vi "GDSAPI_CreateClass.vi"(7 "KeepLvClassRefOpen(False)":bool, 8 "error in (no error)":errorcluster, 9 "ClassIcon(Random colors are used if not wired)":T1, 10 "CreateClassType":T3={"ClassProvider"=enum."GOOP-3(By reference)", "NewClassFolder"=path "", "ParentLvClassFilePath"=path "", "ClassName"="", "ClassDescription"="", "ClassTemplate"=enum."Standard", "ParentInterfacesFilePath"=[]}, 11 "ProjectItemToCreateClassUnder":refnum<vi>) -> (0 "error out":errorcluster, 2 "LVClassLibraryRefnum":refnum<vi>, 3 "LvClassFileOut":path)   [LabVIEW 2020]
doc: "NOT Yet implemented"
uses:
  ClassProviders/Provider_LvNativeClass/ClassWriterNative_class/ClassWriterNative.lvclass
  ClassProviders/Provider_EndevoGOOP300/ClassWriterGOOP300_class/ClassWriterGOOP300.lvclass
  ClassProviders/Provider_EndevoGOOP400/ClassWriterGOOP400_class/ClassWriterGOOP400.lvclass
  ClassProviders/Provider_BaseClassInterface/CreateClassData.ctl
  ClassProviders/Provider_BaseClassInterface/ClassWriter_class/ClassWriter.lvclass
  ClassProviders/Common/ScriptingFunctions/Scripting_ConnectorPanePatternType.ctl
  ClassProviders/Common/LvIcon_class/GDSLvIcon_ClassColorTypes.ctl
  C:/VIT/GitHub/OpenGDS/resource/Framework/Providers/Open_GDS/ClassProviders/Provider_BaseClassInterface/ClassWriter_class/ClassWriter.lvclass
  C:/VIT/GitHub/OpenGDS/resource/Framework/Providers/Open_GDS/ClassProviders/Provider_LvNativeClass/ClassWriterNative_class/ClassWriterNative.lvclass
  C:/VIT/GitHub/OpenGDS/resource/Framework/Providers/Open_GDS/ClassProviders/Provider_EndevoGOOP300/ClassWriterGOOP300_class/ClassWriterGOOP300.lvclass
  C:/VIT/GitHub/OpenGDS/resource/Framework/Providers/Open_GDS/ClassProviders/Provider_EndevoGOOP400/ClassWriterGOOP400_class/ClassWriterGOOP400.lvclass
  GDSAPI_SubVIs/GDSAPI_ClassProviderType.ctl
  GDSAPI_CreateClassType.ctl
  GDSAPI_SubVIs/GDSAPI_ClassTemplateType.ctl
  GDSAPI_SubVIs/GDSAPI_ClassIcon.ctl
  GDSAPI_SubVIs/GDSAPI_ClassIconType.ctl
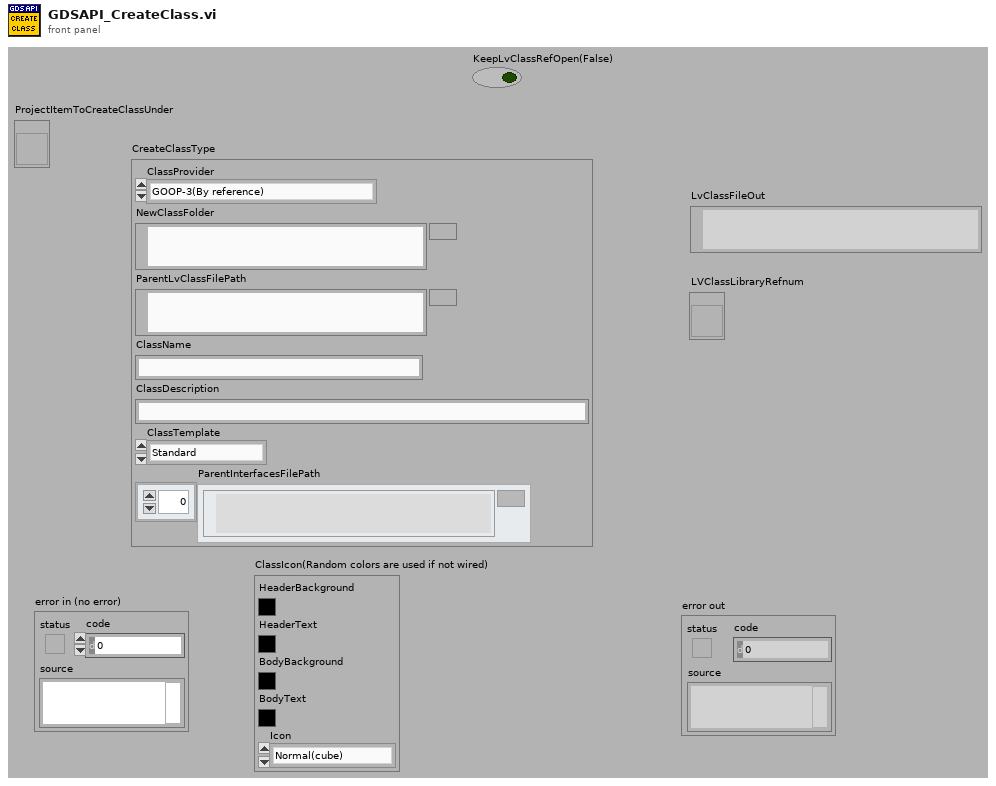
[diagram p1: front panel]
types:
  T1 = typedef "GDSAPI_ClassIcon.ctl" = cluster{"HeaderBackground":u32, "HeaderText":u32, "BodyBackground":u32, "BodyText":u32, "Icon":T2}
  T2 = typedef "GDSAPI_ClassIconType.ctl" = enum16{"Normal(cube)", "Actor", "Message", "Interface"}
  T3 = typedef "GDSAPI_CreateClassType.ctl" = cluster{"ClassProvider":T4, "NewClassFolder":path, "ParentLvClassFilePath":path, "ClassName":string, "ClassDescription":string, "ClassTemplate":T5, "ParentInterfacesFilePath":path[]}
  T4 = typedef "GDSAPI_ClassProviderType.ctl" = enum16{"LabVIEW Native(By value)", "GOOP-3(By reference)", "GOOP-4(By reference)"}
  T5 = typedef "GDSAPI_ClassTemplateType.ctl" = enum16{"Standard", "Singleton"}
  T6 = typedef "GDSLvIcon_ClassColorTypes.ctl" = cluster{"Frame":u32, "Header Text Color":u32, "Header Background":u32, "BodyBackgroundPublic":u32, "BodyBackgroundProtected":u32, "BodyBackgroundPrivate":u32, "Body Text Color":u32, "Frame thickness":u8, "ProtectedPrivateSame":bool, "Icon Header Size":u8, "Font Compression":enum16{"Auto", "On", "Off"}, "CapitalOnly":bool}
  T7 = cluster{"Colors":T6, "LibraryIcon":cluster{"LibraryIcon":string, "HeaderRows(1)":u8}}
  T8 = typedef "ClassWriter.lvclass/CreateClassData.ctl" = cluster{"ClassName":string, "ClassFolder":path, "ClassDescription":string, "ClassTemplateOptions":string, "BaseClass(ProjectStringPath or LvClassFilePath)":variant, "ExtraCreateParameters":variant, "FolderSuffix":string, "ParentInterfaces":path[]}
  T9 = typedef "Scripting_ConnectorPanePatternType.ctl" = u16
  T10 = typedef "GDSLvCLass_ClassSettingsType.ctl" = cluster{"ClassProviderName":string, "ClassTemplateUsed":string, "ClassTemplateVersion":string, "ClassDescription":string, "PlugIns":T11[], "ConnectorPanePattern":string}
  T11 = typedef "GDSLvClass_PlugIn.ctl" = cluster{"Type":T12, "ID":string, "Version":string, "Path":path, "Name":string, "Data":variant}
  T12 = typedef "GDSLvClass_PlugInTypes.ctl" = enum16{"DesignPattern", "MethodTypes"}
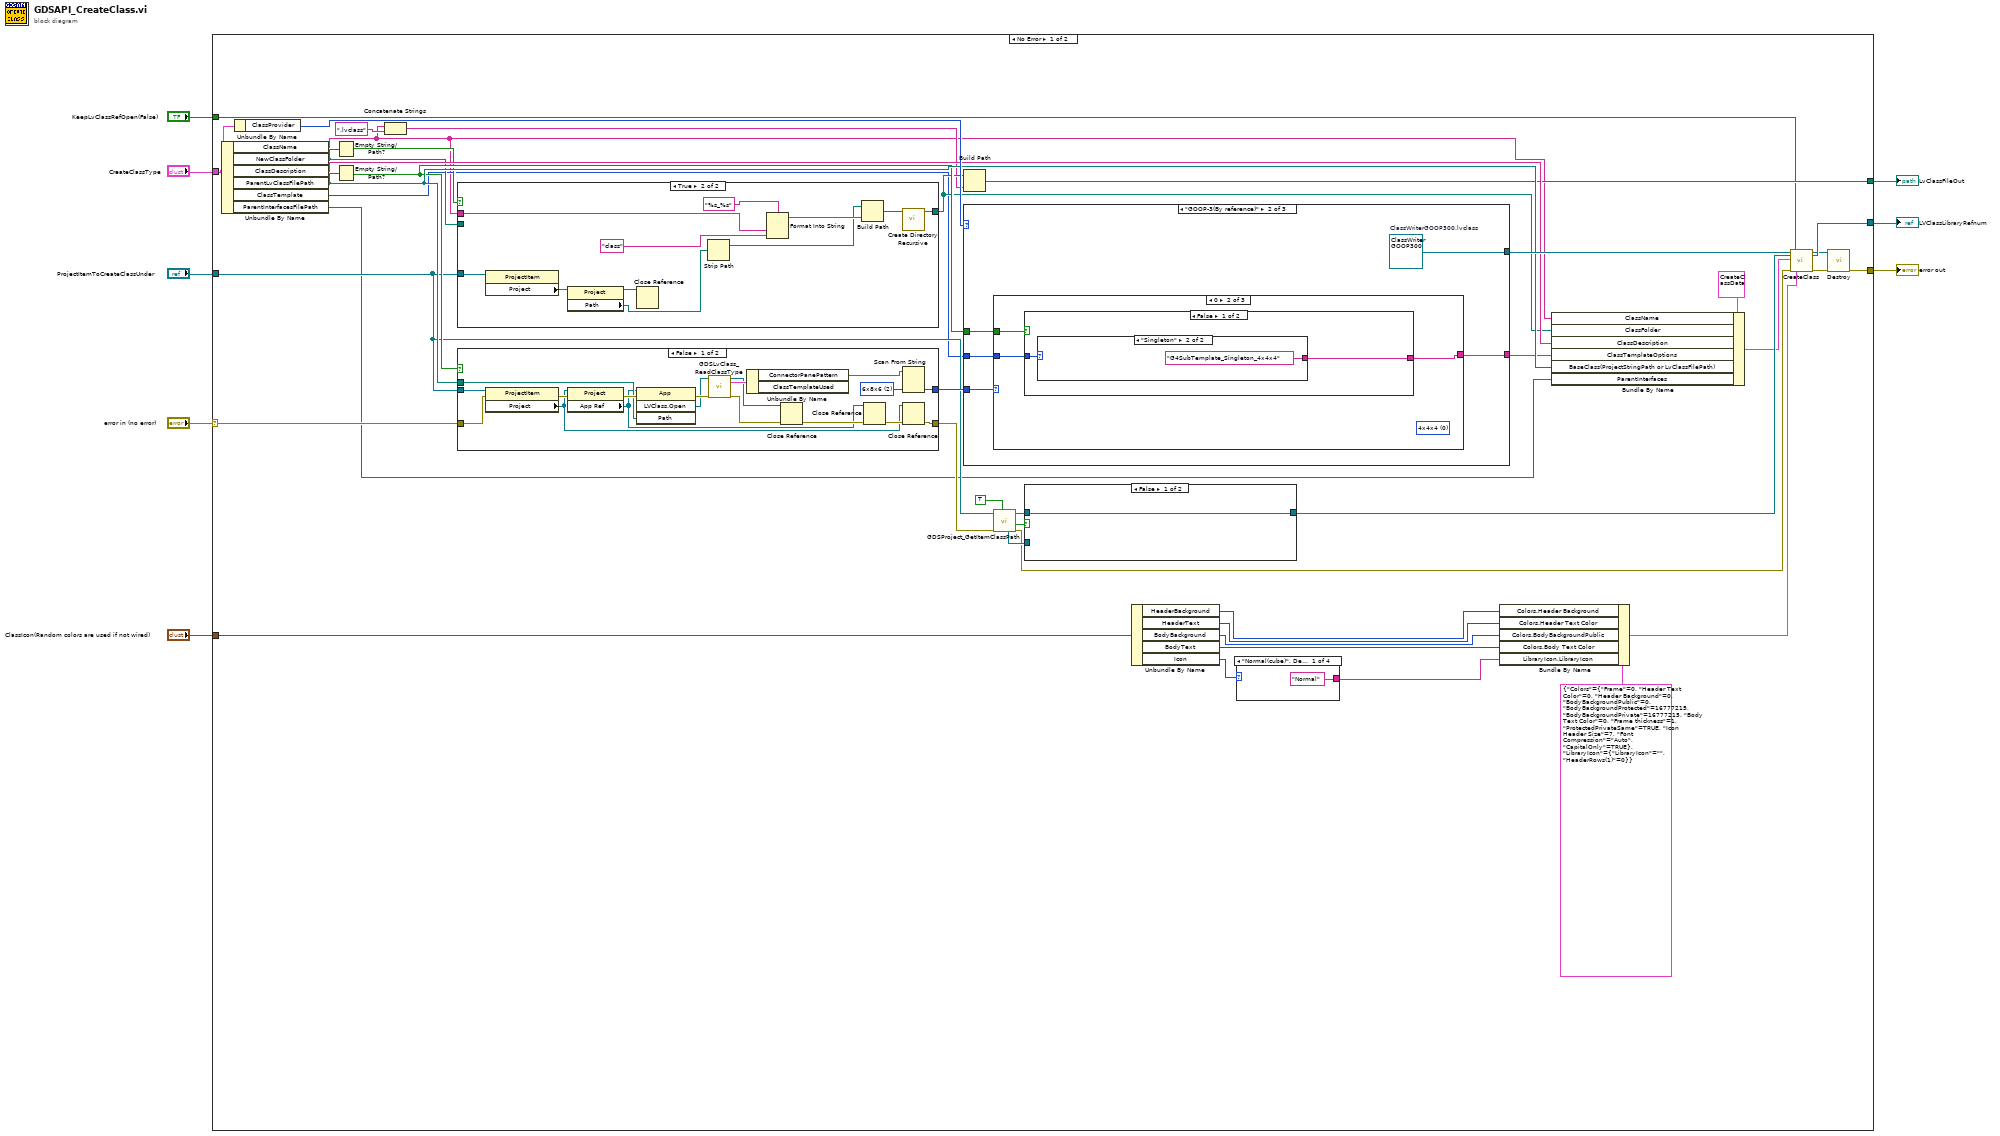
[diagram p0: block diagram]
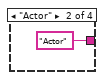
[diagram p2: hidden frame]
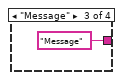
[diagram p3: hidden frame]
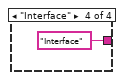
[diagram p4: hidden frame]
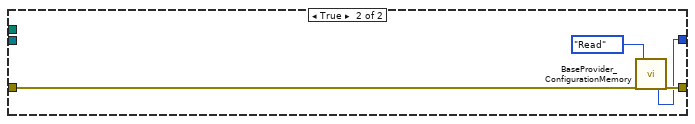
[diagram p6: hidden frame]
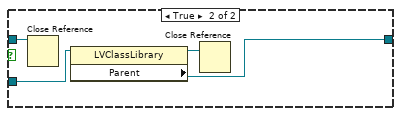
[diagram p7: hidden frame]
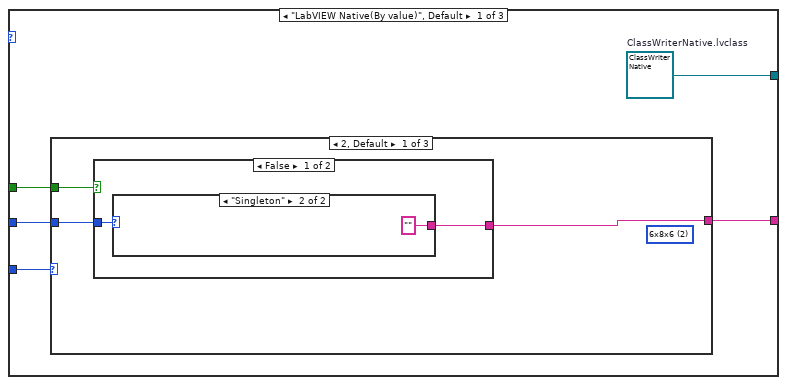
[diagram p8: hidden frame]
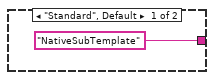
[diagram p9: hidden frame]
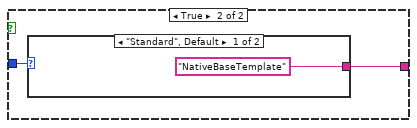
[diagram p10: hidden frame]
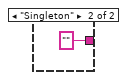
[diagram p11: hidden frame]
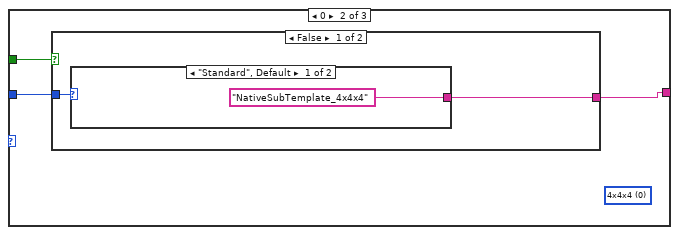
[diagram p12: hidden frame]
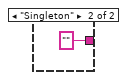
[diagram p13: hidden frame]
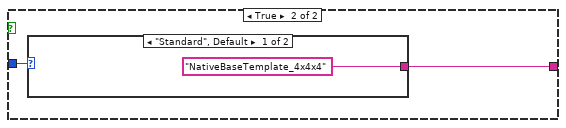
[diagram p14: hidden frame]
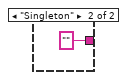
[diagram p15: hidden frame]
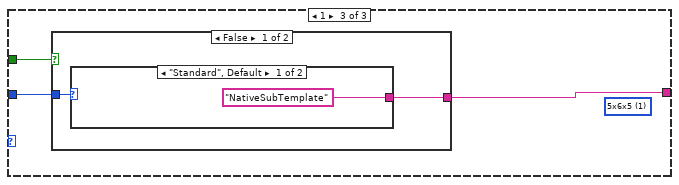
[diagram p16: hidden frame]
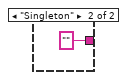
[diagram p17: hidden frame]
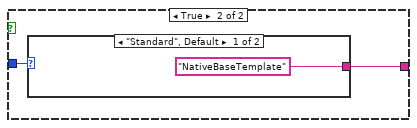
[diagram p18: hidden frame]
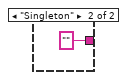
[diagram p19: hidden frame]
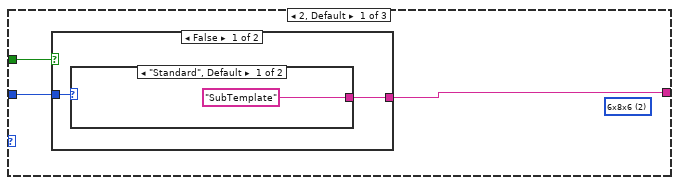
[diagram p20: hidden frame]
diagram:
  n1 = case shown="No Error" "error in (no error)" {
    selector: "error in (no error)" -> [w10 w208]
    tunnel: [w44 _] -> w8
    tunnel: [w40 w208] -> w7
    tunnel: "CreateClassType" -> [w38 _]
    tunnel: "ProjectItemToCreateClassUnder" -> [w29 _]
    tunnel: "ClassIcon(Random colors are used if not wired)" -> [w26 _]
    tunnel: [w16 _] -> w3
    tunnel: "KeepLvClassRefOpen(False)" -> [w11 _]
    frame No Error {
      n2 = Unbundle By Name(w38) -> ("ClassName"=w14:string, "NewClassFolder"=w30:path, "ClassDescription"=w37:string, "ParentLvClassFilePath"=w35:path, "ClassTemplate"=w15:T5, "ParentInterfacesFilePath"=w9:path[])
      n3 = Unbundle By Name(w38) -> ("ClassProvider"=w42:T4)
      n4 = Empty String/Path?(string/path=w30) -> (empty?=w31:bool)
      n5 = Empty String/Path?(string/path=w35) -> (empty?=w33:bool)
      n6 = Concatenate Strings(w14, ".lvclass" ("string")) -> (w17:string)
      n7 = case shown="True" w31 {
        tunnel: w30 -> [w55 _]
        tunnel: [w55 w58] -> w19
        tunnel: w29 -> [_ w66]
        tunnel: w14 -> [_ w56]
        frame False {
        }
        frame True {
          n8 = property class="ProjectItem"(reference=w66) -> ("Project"=w65:refnum<vi>)  [unwired: 1 in, 2 out]
          n9 = property class="Project"(reference=w65) -> (reference out=w63:refnum<vi>, "Path"=w64:path)  [unwired: 1 in, 1 out]
          n10 = Close Reference(reference=w63) -> ()  [unwired: 1 in, 1 out]
          n11 = Strip Path(path=w64) -> (stripped path=w59:path)  [unwired: 1 out]
          n12 = Format Into String(format string="%s_%s", w56, "class" ("format string")) -> (resulting string=w61:string)  [unwired: 2 in, 1 out]
          n13 = Build Path(base path=w59, name or relative path=w61) -> (appended path=w60:path)
          n14 = call <vilib>:"Create Directory Recursive.vi"("directory"=w60) -> ("directory copy"=w58:path)  [unwired: 4 in, 2 out]
        }
      }
      n15 = case shown="False" w33 {
        tunnel: [w67 w87] -> w36
        tunnel: [w81 w86] -> w34
        tunnel: w29 -> [w80 _]
        tunnel: w10 -> [w79 w85]
        tunnel: w35 -> [w74 _]
        frame False {
          w82 = T9 2 items=["4x4x4", "5x6x5", "6x8x6"] ("Pattern")
          n16 = property class="ProjectItem"(reference=w80, error in=w79) -> (error out=w78:errorcluster, "Project"=w69:refnum<vi>)  [unwired: 1 out]
          n17 = property class="Project"(reference=w69, error in=w78) -> (error out=w77:errorcluster, "App Ref"=w71:refnum<vi>)  [unwired: 1 out]
          n18 = invoke class="App" method="LVClass.Open"(reference=w71, error in=w77, "Path"=w74) -> (error out=w76:errorcluster, "LVClass.Open"=w75:refnum<vi>)  [unwired: 1 in, 2 out]
          n19 = call "GDSLvClass_ReadClassType.vi"("Class Refnum In"=w75, "error in (no error)"=w76) -> ("Class Refnum Out"=w73:refnum<vi>, "ClassSettings"=w84:T10, "error out"=w68:errorcluster)  [unwired: 15 in]
          n20 = Unbundle By Name(w84) -> ("ConnectorPanePattern"=w83:string)  [unwired: 1 out]
          n21 = Close Reference(reference=w73, error in (no error)=w68) -> (error out=w72:errorcluster)
          n22 = Close Reference(reference=w71, error in (no error)=w72) -> (error out=w70:errorcluster)
          n23 = Scan From String(input string=w83, default 1=w82) -> (output 1=w81:T9)  [unwired: 3 in, 3 out]
          n24 = Close Reference(reference=w69, error in (no error)=w70) -> (error out=w67:errorcluster)
        }
        frame True {
          n25 = call "BaseProvider_ConfigurationMemory.vi"("error in (no error)"=w85, "Action"=enum16{"Read", "Load", "Save"}."Read") -> ("PatternOut"=w86:T9, "error out"=w87:errorcluster)  [unwired: 11 in, 5 out]
        }
      }
      n26 = Build Path(base path=w19, name or relative path=w17) -> (appended path=w16:path)
      n27 = case shown="\"GOOP-3(By reference)\"" w42 {
        tunnel: [w98 w136 w174] -> w43
        tunnel: w34 -> [w94 w132 w173]
        tunnel: w33 -> [w96 w134 w172]
        tunnel: w15 -> [w95 w133 w171]
        tunnel: [w97 w135 w170] -> w32
        frame "LabVIEW Native(By value)", Default {
          w98 = refnum<class "ClassWriterNative.lvclass"> refnum  # ClassWriterNative.lvclass
          n28 = case shown="2, Default" w94 {
            tunnel: w96 -> [w101 w112 w123]
            tunnel: w95 -> [w100 w111 w122]
            tunnel: [w99 w110 w121] -> w97
            frame 2, Default {
              (unwired) T9 2 items=["4x4x4", "5x6x5", "6x8x6"] ("Pattern")
              n29 = case shown="False" w101 {
                tunnel: w100 -> [w103 w107]
                tunnel: [w102 w106] -> w99
                frame False {
                  n30 = case shown="\"Singleton\"" w103 {
                    tunnel: ["NativeSubTemplate" ("TemplateIdName") "" ("TemplateIdName")] -> w102
                    frame "Standard", Default {
                    }
                    frame "Singleton" {
                    }
                  }
                }
                frame True {
                  n31 = case shown="\"Standard\", Default" w107 {
                    tunnel: ["NativeBaseTemplate" ("TemplateIdName") "" ("TemplateIdName")] -> w106
                    frame "Standard", Default {
                    }
                    frame "Singleton" {
                    }
                  }
                }
              }
            }
            frame 0 {
              (unwired) T9 0 items=["4x4x4", "5x6x5", "6x8x6"] ("Pattern")
              n32 = case shown="False" w112 {
                tunnel: w111 -> [w114 w118]
                tunnel: [w113 w117] -> w110
                frame False {
                  n33 = case shown="\"Standard\", Default" w114 {
                    tunnel: ["NativeSubTemplate_4x4x4" ("TemplateIdName") "" ("TemplateIdName")] -> w113
                    frame "Standard", Default {
                    }
                    frame "Singleton" {
                    }
                  }
                }
                frame True {
                  n34 = case shown="\"Standard\", Default" w118 {
                    tunnel: ["NativeBaseTemplate_4x4x4" ("TemplateIdName") "" ("TemplateIdName")] -> w117
                    frame "Standard", Default {
                    }
                    frame "Singleton" {
                    }
                  }
                }
              }
            }
            frame 1 {
              (unwired) T9 1 items=["4x4x4", "5x6x5", "6x8x6"] ("Pattern")
              n35 = case shown="False" w123 {
                tunnel: w122 -> [w125 w129]
                tunnel: [w124 w128] -> w121
                frame False {
                  n36 = case shown="\"Standard\", Default" w125 {
                    tunnel: ["NativeSubTemplate" ("TemplateIdName") "" ("TemplateIdName")] -> w124
                    frame "Standard", Default {
                    }
                    frame "Singleton" {
                    }
                  }
                }
                frame True {
                  n37 = case shown="\"Standard\", Default" w129 {
                    tunnel: ["NativeBaseTemplate" ("TemplateIdName") "" ("TemplateIdName")] -> w128
                    frame "Standard", Default {
                    }
                    frame "Singleton" {
                    }
                  }
                }
              }
            }
          }
        }
        frame "GOOP-3(By reference)" {
          w136 = refnum<class "ClassWriterGOOP300.lvclass"> refnum  # ClassWriterGOOP300.lvclass
          n38 = case shown="0" w132 {
            tunnel: w134 -> [w139 w150 w161]
            tunnel: w133 -> [w138 w149 w160]
            tunnel: [w137 w148 w159] -> w135
            frame 2, Default {
              (unwired) T9 2 items=["4x4x4", "5x6x5", "6x8x6"] ("Pattern")
              n39 = case shown="False" w139 {
                tunnel: w138 -> [w141 w145]
                tunnel: [w140 w144] -> w137
                frame False {
                  n40 = case shown="\"Standard\", Default" w141 {
                    tunnel: ["SubTemplate" ("TemplateIdName") "" ("TemplateIdName")] -> w140
                    frame "Standard", Default {
                    }
                    frame "Singleton" {
                    }
                  }
                }
                frame True {
                  n41 = case shown="\"Standard\", Default" w145 {
                    tunnel: ["BaseTemplate" ("TemplateIdName") "SingletonTemplate" ("TemplateIdName")] -> w144
                    frame "Standard", Default {
                    }
                    frame "Singleton" {
                    }
                  }
                }
              }
            }
            frame 0 {
              (unwired) T9 0 items=["4x4x4", "5x6x5", "6x8x6"] ("Pattern")
              n42 = case shown="False" w150 {
                tunnel: w149 -> [w152 w156]
                tunnel: [w151 w155] -> w148
                frame False {
                  n43 = case shown="\"Singleton\"" w152 {
                    tunnel: ["SubTemplate_4x4x4" ("TemplateIdName") "G4SubTemplate_Singleton_4x4x4" ("TemplateIdName")] -> w151
                    frame "Standard", Default {
                    }
                    frame "Singleton" {
                    }
                  }
                }
                frame True {
                  n44 = case shown="\"Singleton\"" w156 {
                    tunnel: ["BaseTemplate_4x4x4" ("TemplateIdName") "SingletonTemplate" ("TemplateIdName")] -> w155
                    frame "Standard", Default {
                    }
                    frame "Singleton" {
                    }
                  }
                }
              }
            }
            frame 1 {
              (unwired) T9 1 items=["4x4x4", "5x6x5", "6x8x6"] ("Pattern")
              n45 = case shown="True" w161 {
                tunnel: w160 -> [w163 w167]
                tunnel: [w162 w166] -> w159
                frame False {
                  n46 = case shown="\"Standard\", Default" w163 {
                    tunnel: ["SubTemplate" ("TemplateIdName") "" ("TemplateIdName")] -> w162
                    frame "Standard", Default {
                    }
                    frame "Singleton" {
                    }
                  }
                }
                frame True {
                  n47 = case shown="\"Singleton\"" w167 {
                    tunnel: ["BaseTemplate" ("TemplateIdName") "SingletonTemplate" ("TemplateIdName")] -> w166
                    frame "Standard", Default {
                    }
                    frame "Singleton" {
                    }
                  }
                }
              }
            }
          }
        }
        frame "GOOP-4(By reference)" {
          w174 = refnum<class "ClassWriterGOOP400.lvclass"> refnum  # ClassWriterGOOP400.lvclass
          n48 = case shown="1" w173 {
            tunnel: w172 -> [w177 w188 w199]
            tunnel: w171 -> [w176 w187 w198]
            tunnel: [w175 w186 w197] -> w170
            frame 2, Default {
              (unwired) T9 2 items=["4x4x4", "5x6x5", "6x8x6"] ("Pattern")
              n49 = case shown="False" w177 {
                tunnel: w176 -> [w179 w183]
                tunnel: [w178 w182] -> w175
                frame False {
                  n50 = case shown="\"Singleton\"" w179 {
                    tunnel: ["G4SubTemplate_Simple_6x8x6" ("TemplateIdName") "G4SubTemplate_Singleton_6x8x6" ("TemplateIdName")] -> w178
                    frame "Standard", Default {
                    }
                    frame "Singleton" {
                    }
                  }
                }
                frame True {
                  n51 = case shown="\"Standard\", Default" w183 {
                    tunnel: ["G4BaseTemplate_Simple_6x8x6" ("TemplateIdName") "G4BaseTemplate_Singleton_6x8x6" ("TemplateIdName")] -> w182
                    frame "Standard", Default {
                    }
                    frame "Singleton" {
                    }
                  }
                }
              }
            }
            frame 0 {
              (unwired) T9 0 items=["4x4x4", "5x6x5", "6x8x6"] ("Pattern")
              n52 = case shown="False" w188 {
                tunnel: w187 -> [w190 w194]
                tunnel: [w189 w193] -> w186
                frame False {
                  n53 = case shown="\"Singleton\"" w190 {
                    tunnel: ["G4SubTemplate_Simple_4x4x4" ("TemplateIdName") "G4SubTemplate_Singleton_4x4x4" ("TemplateIdName")] -> w189
                    frame "Standard", Default {
                    }
                    frame "Singleton" {
                    }
                  }
                }
                frame True {
                  n54 = case shown="\"Singleton\"" w194 {
                    tunnel: ["G4BaseTemplate_Simple_4x4x4" ("TemplateIdName") "G4BaseTemplate_Singleton_4x4x4" ("TemplateIdName")] -> w193
                    frame "Standard", Default {
                    }
                    frame "Singleton" {
                    }
                  }
                }
              }
            }
            frame 1 {
              (unwired) T9 1 items=["4x4x4", "5x6x5", "6x8x6"] ("Pattern")
              n55 = case shown="True" w199 {
                tunnel: w198 -> [w201 w205]
                tunnel: [w200 w204] -> w197
                frame False {
                  n56 = case shown="\"Standard\", Default" w201 {
                    tunnel: ["G4SubTemplate_Simple_5x6x5" ("TemplateIdName") "G4SubTemplate_Singleton_5x6x5" ("TemplateIdName")] -> w200
                    frame "Standard", Default {
                    }
                    frame "Singleton" {
                    }
                  }
                }
                frame True {
                  n57 = case shown="\"Standard\", Default" w205 {
                    tunnel: ["G4BaseTemplate_Simple_5x6x5" ("TemplateIdName") "G4BaseTemplate_Singleton_5x6x5" ("TemplateIdName")] -> w204
                    frame "Standard", Default {
                    }
                    frame "Singleton" {
                    }
                  }
                }
              }
            }
          }
        }
      }
      n58 = call "GDSProject_GetItemClassPath.vi"("ReturnRefToClass(False)"=TRUE, "error in"=w36, "ProjectItemRefIn"=w29) -> ("error out"=w41:errorcluster, "LvCLassFound"=w49:bool, "ProjectItemRefOut"=w48:refnum<vi>, "LvClassRef"=w46:refnum<vi>)  [unwired: 3 in, 2 out]
      n59 = case shown="False" w49 {
        tunnel: w48 -> [w89 w93]
        tunnel: [w89 w91] -> w47
        tunnel: w46 -> [_ w92]
        frame False {
        }
        frame True {
          n60 = Close Reference(reference=w93) -> ()  [unwired: 1 in, 1 out]
          n61 = property class="LVClassLibrary"(reference=w92) -> (reference out=w90:refnum<vi>, "Parent"=w91:refnum<vi>)  [unwired: 1 in, 1 out]
          n62 = Close Reference(reference=w90) -> ()  [unwired: 1 in, 1 out]
        }
      }
      n63 = Unbundle By Name(w26) -> ("HeaderBackground"=w25:u32, "HeaderText"=w24:u32, "BodyBackground"=w23:u32, "BodyText"=w22:u32, "Icon"=w21:T2)
      n64 = case shown="\"Normal(cube)\", Default" w21 {
        tunnel: ["Normal" ("LibraryIcon.LibraryIcon") "Actor" "Message" "Interface"] -> w20
        frame "Normal(cube)", Default {
        }
        frame "Actor" {
        }
        frame "Message" {
        }
        frame "Interface" {
        }
      }
      n65 = Bundle By Name(cluster=T7 {"Colors"={"Frame"=0, "Header Text Color"=0, "Header Background"=0, "BodyBackgroundPublic"=0, "BodyBackgroundProtected"=16777215, "BodyBackgroundPrivate"=16777215, "Body Text Color"=0, "Frame thickness"=1, "ProtectedPrivateSame"=TRUE, "Icon Header Size"=7, "Font Compression"=enum."Auto", "CapitalOnly"=TRUE}, "LibraryIcon"={"LibraryIcon"="", "HeaderRows(1)"=0}} ("output cluster"), "Colors.Header Background"=w25, "Colors.Header Text Color"=w24, "Colors.BodyBackgroundPublic"=w23, "Colors.Body Text Color"=w22, "LibraryIcon.LibraryIcon"=w20) -> (w27:T7)
      n66 = Bundle By Name(cluster=T8 {"ClassName"="", "ClassFolder"=path "", "ClassDescription"="", "ClassTemplateOptions"="", "BaseClass(ProjectStringPath or LvClassFilePath)"=variant, "ExtraCreateParameters"=variant, "FolderSuffix"="", "ParentInterfaces"=[]} ("CreateClassData"), "ClassName"=w14, "ClassFolder"=w19, "ClassDescription"=w37, "ClassTemplateOptions"=w32, "BaseClass(ProjectStringPath or LvClassFilePath)"=w35, "ParentInterfaces"=w9) -> (w39:T8)
      n67 = call-dynamic "CreateClass.vi"("ClassWriterNative"=w43, "ProjectTreePosition(String or Project Item Ref)"=w47, "CreateClassData"=w39, "error in (no error)"=w41, "KeepLvClassRefOpen(False)"=w11, "HeaderToApply (take from VIRef or /use 2D-8bit header, Ignored if not wired)"=w27) -> ("ClassWriterNative"=w13:refnum<class "ClassWriterNative.lvclass">, "LVClassLibraryRefnum"=w44:refnum<vi>, "error out"=w45:errorcluster)  [unwired: 10 in, 1 out]
      n68 = call-dynamic "Destroy.vi"("ClassWriterNative"=w13, "error in (no error)"=w45) -> ("error out"=w40:errorcluster)  [unwired: 17 in]
    }
    frame Error {
    }
  }
  "error out" <- w7
  "LvClassFileOut" <- w3
  "LVClassLibraryRefnum" <- w8
